vi "Cascade State Machine.vi"(7 "Description":string, 8 "Command Info In":T2, 11 "Position":T1) -> (0 "Command Info Out":T2)   [LabVIEW 2027]
doc: "This template is useful for immediate subsystem actions that do not need deadband filtering\n\nBe sure to right-click and select New from Template and save with a new command name."
uses:
  <vilib>/Rock Robotics/WPI/Framework/Command Status Info.ctl
  <vilib>/Rock Robotics/WPI/Framework/Completion Status.ctl
  <vilib>/Rock Robotics/WPI/Framework/Completion Notifier.ctl
  Implementation/Cascade Positions.ctl
  Implementation/Cascade Setpoints.ctl
  Implementation/Cascade Operations.ctl
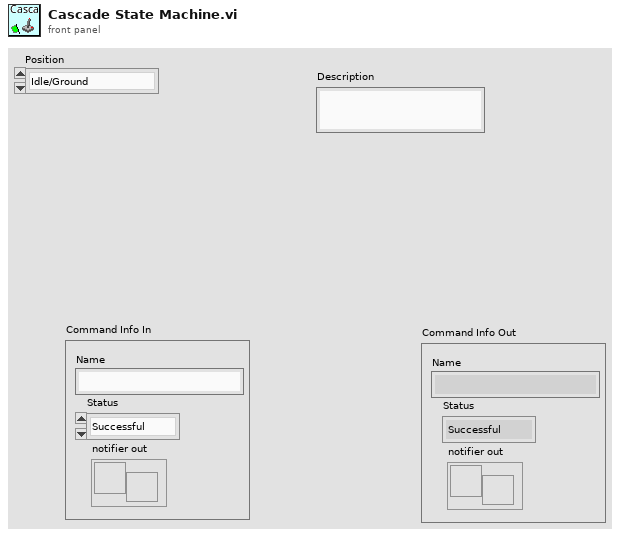
[diagram p1: front panel]
types:
  T1 = typedef "Cascade Positions.ctl" = enum16{"Idle/Ground", "Raised L1", "L2", "L2 Tip", "L3", "L3 Tip", "Feeder", "\"Default\""}
  T2 = typedef "Command Status Info.ctl" = cluster{"Name":string, "Status":T3, "notifier out":T4}
  T3 = typedef "Completion Status.ctl" = enum16{"Successful", "Aborted", "Incomplete"}
  T4 = typedef "Completion Notifier.ctl" = refnum<notifier>
  T5 = typedef "Cascade Setpoints.ctl" = cluster{"Operation":T6, "Position":T1, "Setpoint":dbl}
  T6 = typedef "Cascade Operations.ctl" = enum16{"Reserve", "Read Current", "Immediate", "State Machine"}
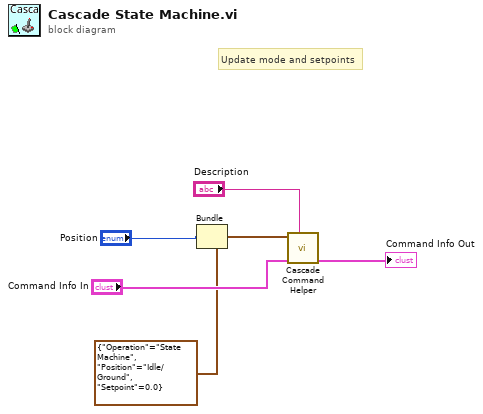
[diagram p0: block diagram]
diagram:
  # "Update mode and setpoints"
  n1 = Bundle(cluster=T5 {"Operation"=enum."State Machine", "Position"=enum."Idle/Ground", "Setpoint"=0.0} ("SubSystem Data"), "Position"="Position") -> (w2:T5)  [unwired: 2 in]
  n2 = call "Cascade Command Helper.vi"("Description"="Description", "Command Info In"="Command Info In", "SubSystem Data"=w2) -> ("Command Info Out"=→"Command Info Out":T2)  [unwired: 6 in, 2 out]
